vi "Run Server.vi"() -> ()   [LabVIEW 2021, in "CanReaderNixnet_server.lvlib"]
uses:
  CanReaderNixnet_server.lvlib
  <vilib>/gRPC/LabVIEW gRPC Servicer/ServiceBase/ServiceBase.lvclass
  <vilib>/gRPC/LabVIEW gRPC Servicer/Servicer/Servicer.lvclass
panel:
  in  "Async [T] / Sync [F]":bool
  out "Listening Port":i32
  in  "Stop":bool
  in  "Server Address":string="localhost:50051"
  in  "Server Certificate File (.crt)":path
  in  "Server Key File (.key)":path
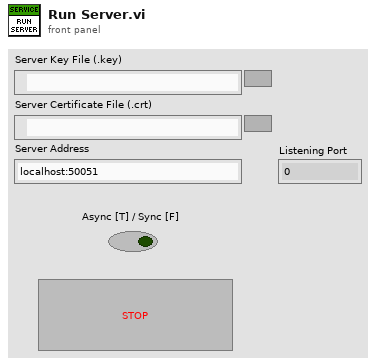
[diagram p1: front panel]
types:
  T1 = enum32{"Invalid", "Standard", "Closed", "Hidden", "Minimized", "Maximized"}
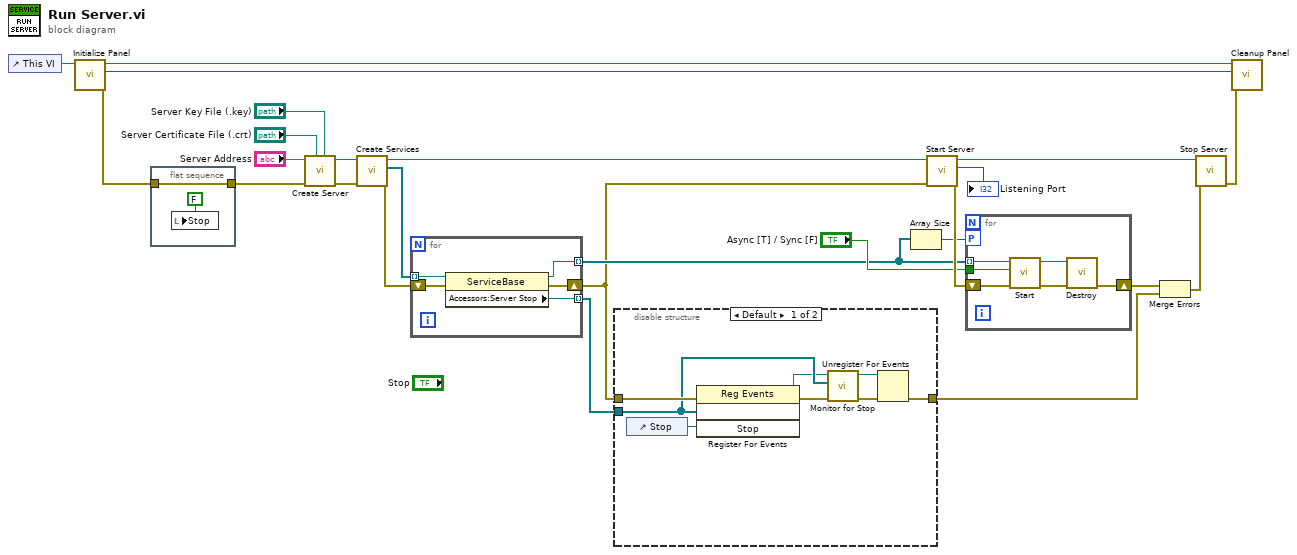
[diagram p0: block diagram]
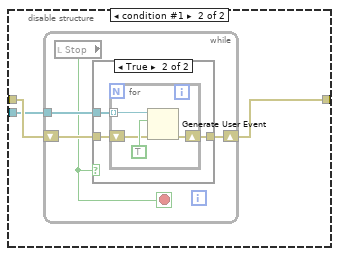
[diagram p2: hidden frame]
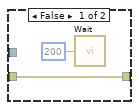
[diagram p3: hidden frame]
diagram:
  n1 = control-ref of="This VI"() -> (w10:refnum<vi>)
  n2 = call "Initialize Panel.vi"("vi reference in"=w10) -> ("error out"=w3:errorcluster, "initial window state"=w8:T1, "vi reference out"=w9:refnum<vi>)  [unwired: 8 in]
  n3 = flat-sequence {
    tunnel: w3 -> [w27]
    tunnel: [w27] -> w2
    frame #0 {
      n4 = local write "Stop"(FALSE ("Stop")) -> ()
    }
  }
  n5 = call <vilib>:"Create Server.vi"("Server Key File (.key)"="Server Key File (.key)", "Server Certificate File (.crt)"="Server Certificate File (.crt)", "error in"=w2, "Server Address"="Server Address") -> ("error out"=w6:errorcluster, "gRPC server out"=w20:refnum<class "Servicer.lvclass">)  [unwired: 6 in]
  n6 = call "Create Services.vi"("error in (no error)"=w6, "gRPC server in"=w20) -> ("error out"=w5:errorcluster, "gRPC services out"=w4:refnum<class "ServiceBase.lvclass">[], "gRPC server out"=w19:refnum<class "Servicer.lvclass">)  [unwired: 7 in]
  n7 = for {
    tunnel: [w31] -> w14 mode=indexing
    shift-right: [w30] -> w1
    shift-left: w5 -> [w28]
    tunnel: [w32] -> w15 mode=indexing
    tunnel: w4 -> [w29] mode=indexing
    n8 = property class="ServiceBase"(reference=w29, error in=w28) -> (reference out=w32:refnum<class "ServiceBase.lvclass">, error out=w30:errorcluster, "Accessors:Server Stop"=w31:refnum<user-event>)
  }
  n9 = disable-structure shown="Default" {
    disable-tunnel: w14 -> [w35 w42]
    disable-tunnel: w1 -> [w40 w43]
    disable-tunnel: [w33 w41] -> w13
    frame condition #0 (active) {
      n10 = control-ref of="Stop"() -> (w39:refnum<vi>)
      n11 = register-events(error in=w40, w35, w39) -> (reference out=w34:refnum<event-registration>, error out=w36:errorcluster)  [unwired: 1 in]
      n12 = call "Monitor for Stop.vi"("error in (no error)"=w36, "service stop events"=w35, "Event Registration Refnum"=w34) -> ("error out"=w37:errorcluster, "Event Registration Refnum"=w38:refnum<event-registration>)  [unwired: 7 in]
      n13 = Unregister For Events(event registration refnum=w38, error in=w37) -> (error out=w33:errorcluster)
    }
    frame condition #1 {
      n14 = while {
        tunnel: w42 -> [w46]
        shift-right: [w45] -> w41
        shift-left: w43 -> [w47]
        stop <- w44 stop-if-true
        n15 = local read "Stop"() -> (w44:bool)
        n16 = case shown="True" w44 {
          tunnel: [w49 w52] -> w45
          tunnel: w47 -> [w49 w50]
          tunnel: w46 -> [_ w51]
          frame False {
            n17 = call "Wait"("Count(mSec)"=u32 200) -> ()  [unwired: 1 out]
          }
          frame True {
            n18 = for {
              shift-right: [w54] -> w52
              shift-left: w50 -> [w55]
              tunnel: w51 -> [w53] mode=indexing
              n19 = Generate User Event(user event=w53, event data cluster=TRUE ("event data"), error in=w55) -> (error out=w54:errorcluster)  [unwired: 1 in, 1 out]
            }
          }
        }
      }
    }
  }
  n20 = Array Size(array=w15) -> (size(s)=w16:i32)
  n21 = call <vilib>:"Start Server.vi"("error in"=w1, "gRPC server in"=w19) -> ("error out"=w18:errorcluster, "Listening Port"=→"Listening Port":i32, "gRPC server out"=w25:refnum<class "Servicer.lvclass">)  [unwired: 7 in]
  n22 = for {
    tunnel: w15 -> [w60] mode=indexing
    tunnel: "Async [T] / Sync [F]" -> [w58]
    workers-P: w16 -> [_]
    shift-right: [w57] -> w12
    shift-left: w18 -> [w59]
    n23 = call-dynamic "Start.vi"("error in"=w59, "ASync [T]"=w58, "gRPC service in"=w60) -> ("error out"=w61:errorcluster, "gRPC service out"=w62:refnum<class "ServiceBase.lvclass">)  [unwired: 7 in]
    n24 = call-dynamic "Destroy.vi"("error in"=w61, "gRPC service in"=w62) -> ("error out"=w57:errorcluster)  [unwired: 8 in, 1 out]
  }
  n25 = Merge Errors(w12, w13) -> (w11:errorcluster)
  n26 = call <vilib>:"Stop Server.vi"("error in"=w11, "gRPC server in"=w25) -> ("error out"=w7:errorcluster)  [unwired: 9 in]
  n27 = call "Cleanup Panel.vi"("error in (no error)"=w7, "initial window state"=w8, "vi reference in"=w9) -> ()  [unwired: 7 in, 2 out]
